vi "Func - FuncVI Refnums (Open Master).vi"(7 "Func Info in":T1, 8 "error in":errorcluster, 9 "open CSE FuncVI2 (F)":bool, 11 "Func name":string) -> (0 "error out":errorcluster, 2 "FuncVI2 RefNum":refnum<vi>, 3 "FuncVI RefNum":refnum<vi>, 5 "Func Info out":T1)   [LabVIEW 2021]
doc: "::: CalcExpress Toolkit :::\nCopyright (c) 2000-2026 Konstantin Shifershteyn. All rights reserved."
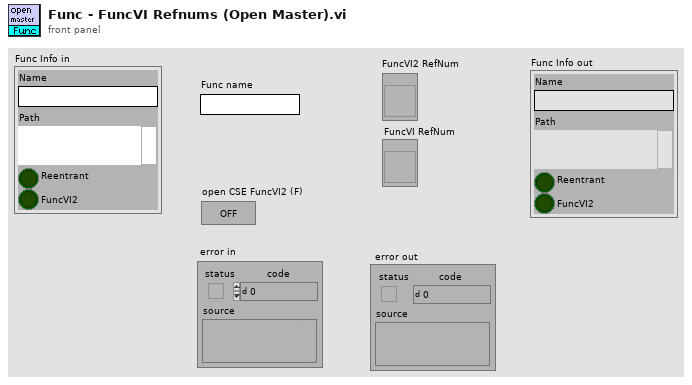
[diagram p1: front panel]
types:
  T1 = cluster{"Name":string, "Path":path, "Reentrant":bool, "FuncVI2":bool}
  T2 = cluster{"Name":string, "Path":path, "Exec.IsReentrant":bool, bool}
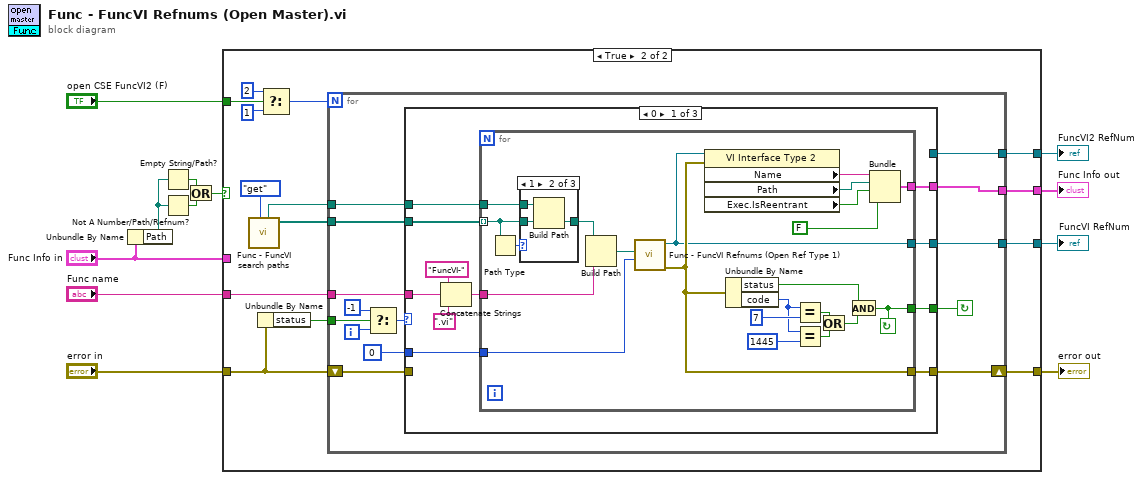
[diagram p0: block diagram]
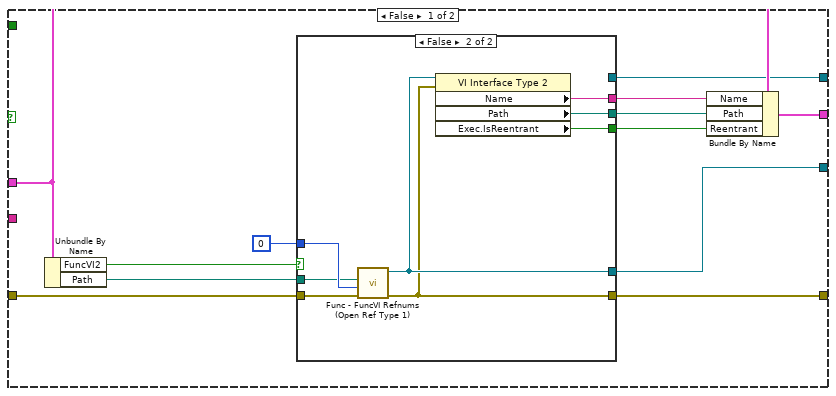
[diagram p2: hidden frame]
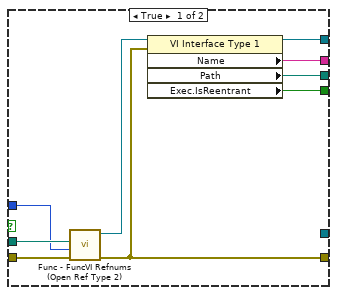
[diagram p3: hidden frame]
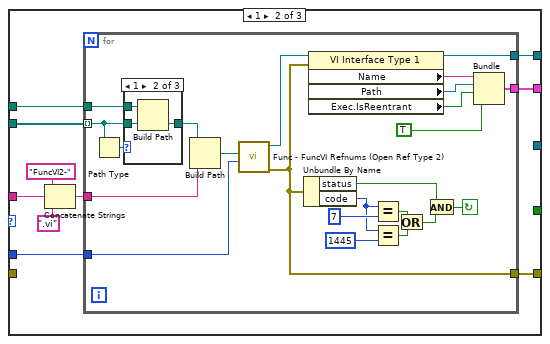
[diagram p6: hidden frame]
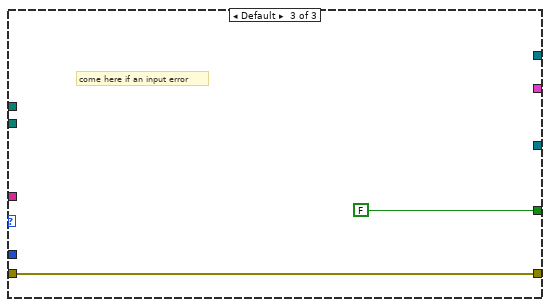
[diagram p9: hidden frame]
diagram:
  n1 = Unbundle By Name("Func Info in") -> ("Path"=w5:path)
  n2 = Empty String/Path?(string/path=w5) -> (empty?=w9:bool)
  n3 = Not A Number/Path/Refnum?(number/path/refnum=w5) -> (NaN/Path/Refnum?=w10:bool)
  n4 = Or(x=w9, y=w10) -> (x .or. y?=w7:bool)
  n5 = case shown="True" w7 {
    tunnel: [w13 w52] -> w12
    tunnel: [w21 w51] -> w11
    tunnel: [w18 w50] -> w2
    tunnel: "error in" -> [w22 w43]
    tunnel: [w24 w49] -> w6
    tunnel: "open CSE FuncVI2 (F)" -> [_ w48]
    tunnel: "Func Info in" -> [w23 _]
    tunnel: "Func name" -> [_ w44]
    frame False {
      n6 = Unbundle By Name(w23) -> ("FuncVI2"=w19:bool, "Path"=w20:path)
      n7 = case shown="False" w19 {
        tunnel: w22 -> [w27 w36]
        tunnel: [w25 w34] -> w21
        tunnel: w20 -> [w29 w37]
        tunnel: [w33 _] -> w18
        tunnel: [w32 w41] -> w17
        tunnel: [w31 w40] -> w16
        tunnel: [w30 w39] -> w15
        tunnel: 0 ("options") -> [w28 w38]
        tunnel: [_ w35] -> w13
        frame True {
          n8 = call "Func - FuncVI Refnums (Open Ref Type 2).vi"("error in"=w27, "options"=w28, "vi path"=w29) -> ("error out"=w25:errorcluster, "FuncVI2 RefNum"=w26:refnum<vi>)  [unwired: 7 in]
          n9 = property on="Property Node" class="VI Interface Type 1"(reference=w26, error in=w25) -> (reference out=w33:refnum<vi>, "Name"=w32:string, "Path"=w31:path, "Exec.IsReentrant"=w30:bool)  [unwired: 1 out]
        }
        frame False {
          n10 = call "Func - FuncVI Refnums (Open Ref Type 1).vi"("error in"=w36, "options"=w38, "vi path"=w37) -> ("error out"=w34:errorcluster, "FuncVI RefNum"=w35:refnum<vi>)  [unwired: 7 in]
          n11 = property on="Property Node" class="VI Interface Type 2"(reference=w35, error in=w34) -> ("Name"=w41:string, "Path"=w40:path, "Exec.IsReentrant"=w39:bool)  [unwired: 2 out]
        }
      }
      n12 = Bundle By Name(cluster=w23, "Name"=w17, "Path"=w16, "Reentrant"=w15) -> (w24:T1)
    }
    frame True {
      n13 = call "Func - FuncVI search paths.vi"("cmd"=enum16{"get", "set"}."get") -> ("search paths"=w53:path[], "base path"=w54:path)  [unwired: 5 in, 2 out]
      n14 = Unbundle By Name(w43) -> ("status"=w42:bool)
      n15 = Select(t=2, s=w48, f=1) -> (s? t:f=w45:i32)
      n16 = for {
        N: w45 -> [_]
        tunnel: [w66] -> w52
        tunnel: w44 -> [w67]
        tunnel: w53 -> [w68]
        tunnel: w54 -> [w69]
        tunnel: [w64] -> w50
        tunnel: [w63] -> w49
        tunnel: w42 -> [w59]
        shift-right: [w65] -> w51
        shift-left: w43 -> [w56]
        i -> [w60]
        stop <- w62 continue-if-true
        n17 = Select(t=-1, s=w59, f=w60) -> (s? t:f=w58:i32)
        n18 = case shown="0" w58 {
          tunnel: w69 -> [w80 w117 _]
          tunnel: w68 -> [w79 w116 _]
          tunnel: w67 -> [w77 w114 _]
          tunnel: [w76 _ _] -> w66
          tunnel: [w75 _ FALSE] -> w62
          tunnel: [w74 w113 w146] -> w65
          tunnel: [_ w110 _] -> w64
          tunnel: [w71 w109 _] -> w63
          tunnel: w56 -> [_ _ w146]
          tunnel: 0 ("options") -> [w70 w108 _]
          frame 0 {
            n19 = Concatenate Strings("FuncVI-", w77, ".vi" ("func name")) -> (w78:string)
            n20 = for {
              tunnel: [w95] -> w75
              tunnel: [w86] -> w76
              tunnel: [w87] -> w74
              tunnel: w80 -> [w100]
              tunnel: w79 -> [w102] mode=indexing
              tunnel: w78 -> [w98]
              tunnel: [w91] -> w71
              tunnel: w70 -> [w89]
              stop <- w95 continue-if-true
              n21 = Path Type(1:w102) -> (0:w101:i16)
              n22 = case shown="1" w101 {
                tunnel: w102 -> [w103 w105 w107]
                tunnel: w100 -> [_ w106 _]
                tunnel: [w103 w104 w107] -> w99
                frame ..0 {
                }
                frame 1 {
                  n23 = Build Path(base path=w106, name or relative path=w105) -> (appended path=w104:path)
                }
                frame 2.. {
                }
              }
              n24 = Build Path(base path=w99, name or relative path=w98) -> (appended path=w88:path)
              n25 = call "Func - FuncVI Refnums (Open Ref Type 1).vi"("options"=w89, "vi path"=w88) -> ("error out"=w87:errorcluster, "FuncVI RefNum"=w86:refnum<vi>)  [unwired: 8 in]
              n26 = property on="Property Node" class="VI Interface Type 2"(reference=w86, error in=w87) -> ("Name"=w93:string, "Path"=w94:path, "Exec.IsReentrant"=w92:bool)  [unwired: 2 out]
              n27 = Unbundle By Name(w87) -> ("status"=w96:bool, "code"=w85:i32)
              n28 = Equal?(x=w85, y=7) -> (x = y?=w83:bool)
              n29 = Equal?(x=w85, y=1445) -> (x = y?=w82:bool)
              n30 = Or(x=w83, y=w82) -> (x .or. y?=w81:bool)
              n31 = And(x=w96, y=w81) -> (x .and. y?=w95:bool)
              n32 = Bundle("Name"=w93, "Path"=w94, "Exec.IsReentrant"=w92, FALSE) -> (w91:T2)  [unwired: 1 in]
            }
          }
          frame 1 {
            n33 = Concatenate Strings("FuncVI2-", w114, ".vi" ("func name")) -> (w115:string)
            n34 = for {
              tunnel: [w119] -> w113
              tunnel: w117 -> [w138]
              tunnel: w116 -> [w140] mode=indexing
              tunnel: w115 -> [w136]
              tunnel: [w135] -> w110
              tunnel: [w131] -> w109
              tunnel: w108 -> [w128]
              stop <- w118 continue-if-true
              n35 = Path Type(1:w140) -> (0:w139:i16)
              n36 = case shown="1" w139 {
                tunnel: w140 -> [w141 w143 w145]
                tunnel: w138 -> [_ w144 _]
                tunnel: [w141 w142 w145] -> w137
                frame ..0 {
                }
                frame 1 {
                  n37 = Build Path(base path=w144, name or relative path=w143) -> (appended path=w142:path)
                }
                frame 2.. {
                }
              }
              n38 = Build Path(base path=w137, name or relative path=w136) -> (appended path=w129:path)
              n39 = call "Func - FuncVI Refnums (Open Ref Type 2).vi"("options"=w128, "vi path"=w129) -> ("error out"=w119:errorcluster, "FuncVI2 RefNum"=w127:refnum<vi>)  [unwired: 8 in]
              n40 = Unbundle By Name(w119) -> ("status"=w125:bool, "code"=w124:i32)
              n41 = property on="Property Node" class="VI Interface Type 1"(reference=w127, error in=w119) -> (reference out=w135:refnum<vi>, "Name"=w133:string, "Path"=w134:path, "Exec.IsReentrant"=w132:bool)  [unwired: 1 out]
              n42 = Equal?(x=w124, y=7) -> (x = y?=w122:bool)
              n43 = Equal?(x=w124, y=1445) -> (x = y?=w121:bool)
              n44 = Or(x=w122, y=w121) -> (x .or. y?=w120:bool)
              n45 = And(x=w125, y=w120) -> (x .and. y?=w118:bool)
              n46 = Bundle("Name"=w133, "Path"=w134, "Exec.IsReentrant"=w132, TRUE) -> (w131:T2)  [unwired: 1 in]
            }
          }
          frame Default {
            # "come here if an input error"
          }
        }
      }
    }
  }
  "error out" <- w11
  "FuncVI RefNum" <- w12
  "FuncVI2 RefNum" <- w2
  "Func Info out" <- w6
